vi "mupGetExprVars.vi"(8 "error in (no error)":errorcluster, 11 "hParser in":u64) -> (0 "error out":errorcluster, 1 "varAddrs":u64[](array[numeric]), 2 "varNames":string[](array[string]), 3 "hParser out":u64, 5 "numVars":i32)   [LabVIEW 2018, in "mupLib.lvlib"]
doc: "Reads the list of variable names and pointers that have been defined on this muParser instance."
uses:
  mupLib.lvlib
  <vilib>/Utility/error.llb/Error Cluster From Error Code.vi
  libmuparser-lv.dll
panel:
  # "Reads the list of variable names and pointers that have been defined on this muParser instance."
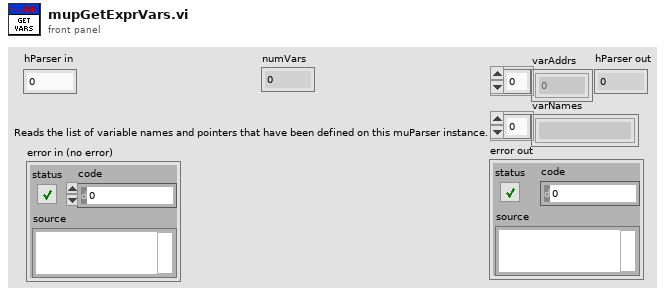
[diagram p1: front panel]
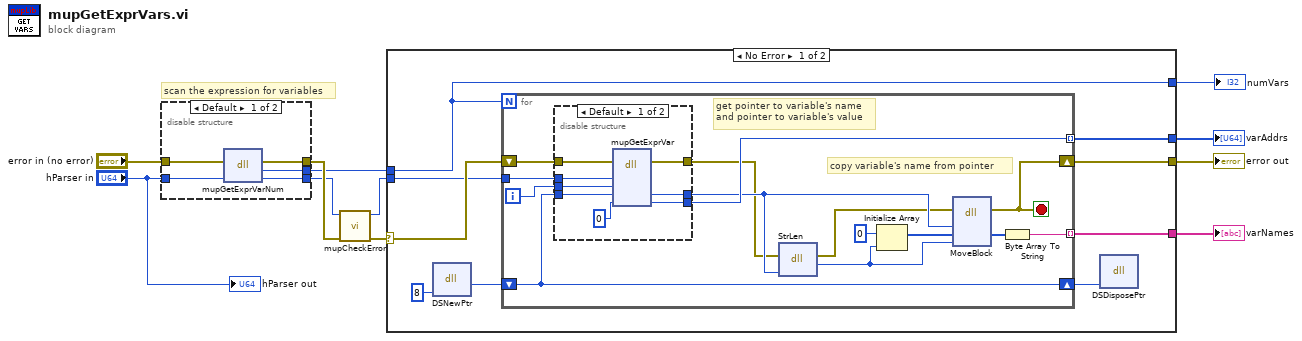
[diagram p0: block diagram]
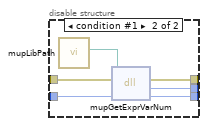
[diagram p2: hidden frame]
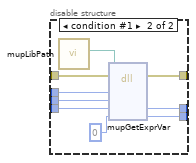
[diagram p3: hidden frame]
diagram:
  # "scan the expression for variables"
  n1 = disable-structure shown="Default" {
    disable-tunnel: [w16 w22] -> w11
    disable-tunnel: [w15 w21] -> w10
    disable-tunnel: "error in (no error)" -> [w14 w20]
    disable-tunnel: "hParser in" -> [w13 w19]
    disable-tunnel: [w12 w18] -> w2
    frame condition #0 (active) {
      n2 = dll-call lib="C:/Users/leonidas/Documents/GitHub/LV-muParser/mupLib/libmuparser-lv.dll" fn="mupGetExprVarNum"(error in=w14, "hParser"=w13) -> (error out=w16:errorcluster, "return type"=w15:i32, "hParser"=w12:u64)  [unwired: 2 in, 1 out]
    }
    frame condition #1 {
      n3 = call "mupLibPath.vi"() -> ("libmuparser path"=w17:path)  [unwired: 11 in]
      n4 = dll-call lib="C:/Users/leonidas/Documents/GitHub/LV-muParser/mupLib/libmuparser-lv.dll" fn="mupGetExprVarNum"(path in=w17, error in=w20, "hParser"=w19) -> (error out=w22:errorcluster, "return type"=w21:i32, "hParser"=w18:u64)  [unwired: 1 in, 1 out]
    }
  }
  n5 = call "mupCheckError.vi"("error in (no error)"=w11, "hParser in"=w2) -> ("error out"=w5:errorcluster, "hParser out"=w1:u64)  [unwired: 8 in]
  n6 = case shown="No Error" w5 {
    selector: w5 -> [w25 w63]
    tunnel: w10 -> [w24 _]
    tunnel: [w29 _] -> w9
    tunnel: [w28 _] -> w8
    tunnel: [w27 w63] -> w7
    tunnel: [w24 _] -> w4
    tunnel: w1 -> [w23 _]
    frame No Error {
      n7 = dll-call lib="LabVIEW" fn="DSNewPtr"("size"=8) -> ("return type"=w30:u64)  [unwired: 4 in, 2 out]
      n8 = for {
        N: w24 -> [_]
        shift-right: [w41] -> w27
        shift-left: w25 -> [w44]
        tunnel: [w40] -> w28 mode=indexing
        tunnel: [w42] -> w29 mode=indexing
        shift-right: [w35] -> w26
        shift-left: w30 -> [w35]
        tunnel: w23 -> [w45]
        i -> [w43]
        stop <- w41 stop-if-true
        # "copy variable's name from pointer"
        # "get pointer to variable's name\nand pointer to variable's value"
        n9 = disable-structure shown="Default" {
          disable-tunnel: w45 -> [w53 w62]
          disable-tunnel: w44 -> [w51 w60]
          disable-tunnel: w43 -> [w50 w59]
          disable-tunnel: [w49 w58] -> w42
          disable-tunnel: [w48 w57] -> w39
          disable-tunnel: [w47 w56] -> w37
          disable-tunnel: w35 -> [w46 w55]
          frame condition #0 (active) {
            n10 = dll-call lib="C:/Users/leonidas/Documents/GitHub/LV-muParser/mupLib/libmuparser-lv.dll" fn="mupGetExprVar"(error in=w51, "hParser"=w53, "varNum"=w50, "varName"=w46, "varAddr"=u64 0) -> (error out=w47:errorcluster, "varName"=w48:u64, "varAddr"=w49:u64)  [unwired: 5 in, 1 out]
          }
          frame condition #1 {
            n11 = call "mupLibPath.vi"() -> ("libmuparser path"=w54:path)  [unwired: 11 in]
            n12 = dll-call lib="C:/Users/leonidas/Documents/GitHub/LV-muParser/mupLib/libmuparser-lv.dll" fn="mupGetExprVar"(path in=w54, error in=w60, "hParser"=w62, "varNum"=w59, "varName"=w55, "varAddr"=u64 0) -> (error out=w56:errorcluster, "varName"=w57:u64, "varAddr"=w58:u64)  [unwired: 4 in, 1 out]
          }
        }
        n13 = dll-call lib="LabVIEW" fn="StrLen"(error in=w37, "pointer"=w39) -> (error out=w36:errorcluster, "return type"=w38:i32)  [unwired: 3 in, 1 out]
        n14 = Initialize Array(u8 0 ("Numeric"), w38) -> (w33:u8[])
        n15 = dll-call lib="LabVIEW" fn="MoveBlock"(error in=w36, "ps"=w39, "pd"=w33, "size"=w38) -> (error out=w41:errorcluster, "pd"=w32:u8[])  [unwired: 5 in, 1 out]
        n16 = Byte Array To String(unsigned byte array=w32) -> (string=w40:string)
      }
      n17 = dll-call lib="LabVIEW" fn="DSDisposePtr"("ptr"=w26) -> ()  [unwired: 5 in, 2 out]
    }
    frame Error {
    }
  }
  "varAddrs" <- w9
  "varNames" <- w8
  "error out" <- w7
  "numVars" <- w4
  "hParser out" <- "hParser in"
